vi "Parameter selection.vi"(2 "Selected Channel":i32(listbox), 5 "Hc0 2":i32(listbox), 7 "默认":bool=TRUE, 10 "全部结构组":T1[](array[typedef]), 11 "逻辑通道组":i32[](array[numeric])) -> (0 "subarray":string[](array[string]), 1 "改变？":bool, 3 "通道组":i32[](array[numeric]), 4 "Array 2":string[](array[string]))   [LabVIEW 2025]
uses:
  data structure.ctl
panel:
  out "Array 6":string[](array[string])
  out "Array":string[](array[string])
  out "subarray 4":string[](array[string])
  out "subarray 3":string[](array[string])
  out "deleted portion":string[](array[string])
  out "subarray 2":string[](array[string])
  out "Array 5":string[][](array[string])
  out "array w/ subset deleted":string[][](array[string])
  out "Array 4":string[](array[string])
  out "Array 3":string[](array[string])
  out "Item Names 2":string[][](array[string])
  in  "数据列表 2":enum32{"40TR", "Chiller"}(tab)
  in  "Hc1 2":i32(listbox)
  in  "数据列表":enum32{"40TR", "Chiller"}(tab)
  in  "Hc0":i32(listbox)
  in  "Hc1":i32(listbox)
  out "Item Names":string[][](array[string])
  in  "取消按钮":bool
  in  "确定按钮":bool
  in  "向下按钮":bool
  in  "向上按钮":bool
  in  "删除按钮":bool
  in  "添加按钮":bool
  in  "All Channel":i32(listbox)
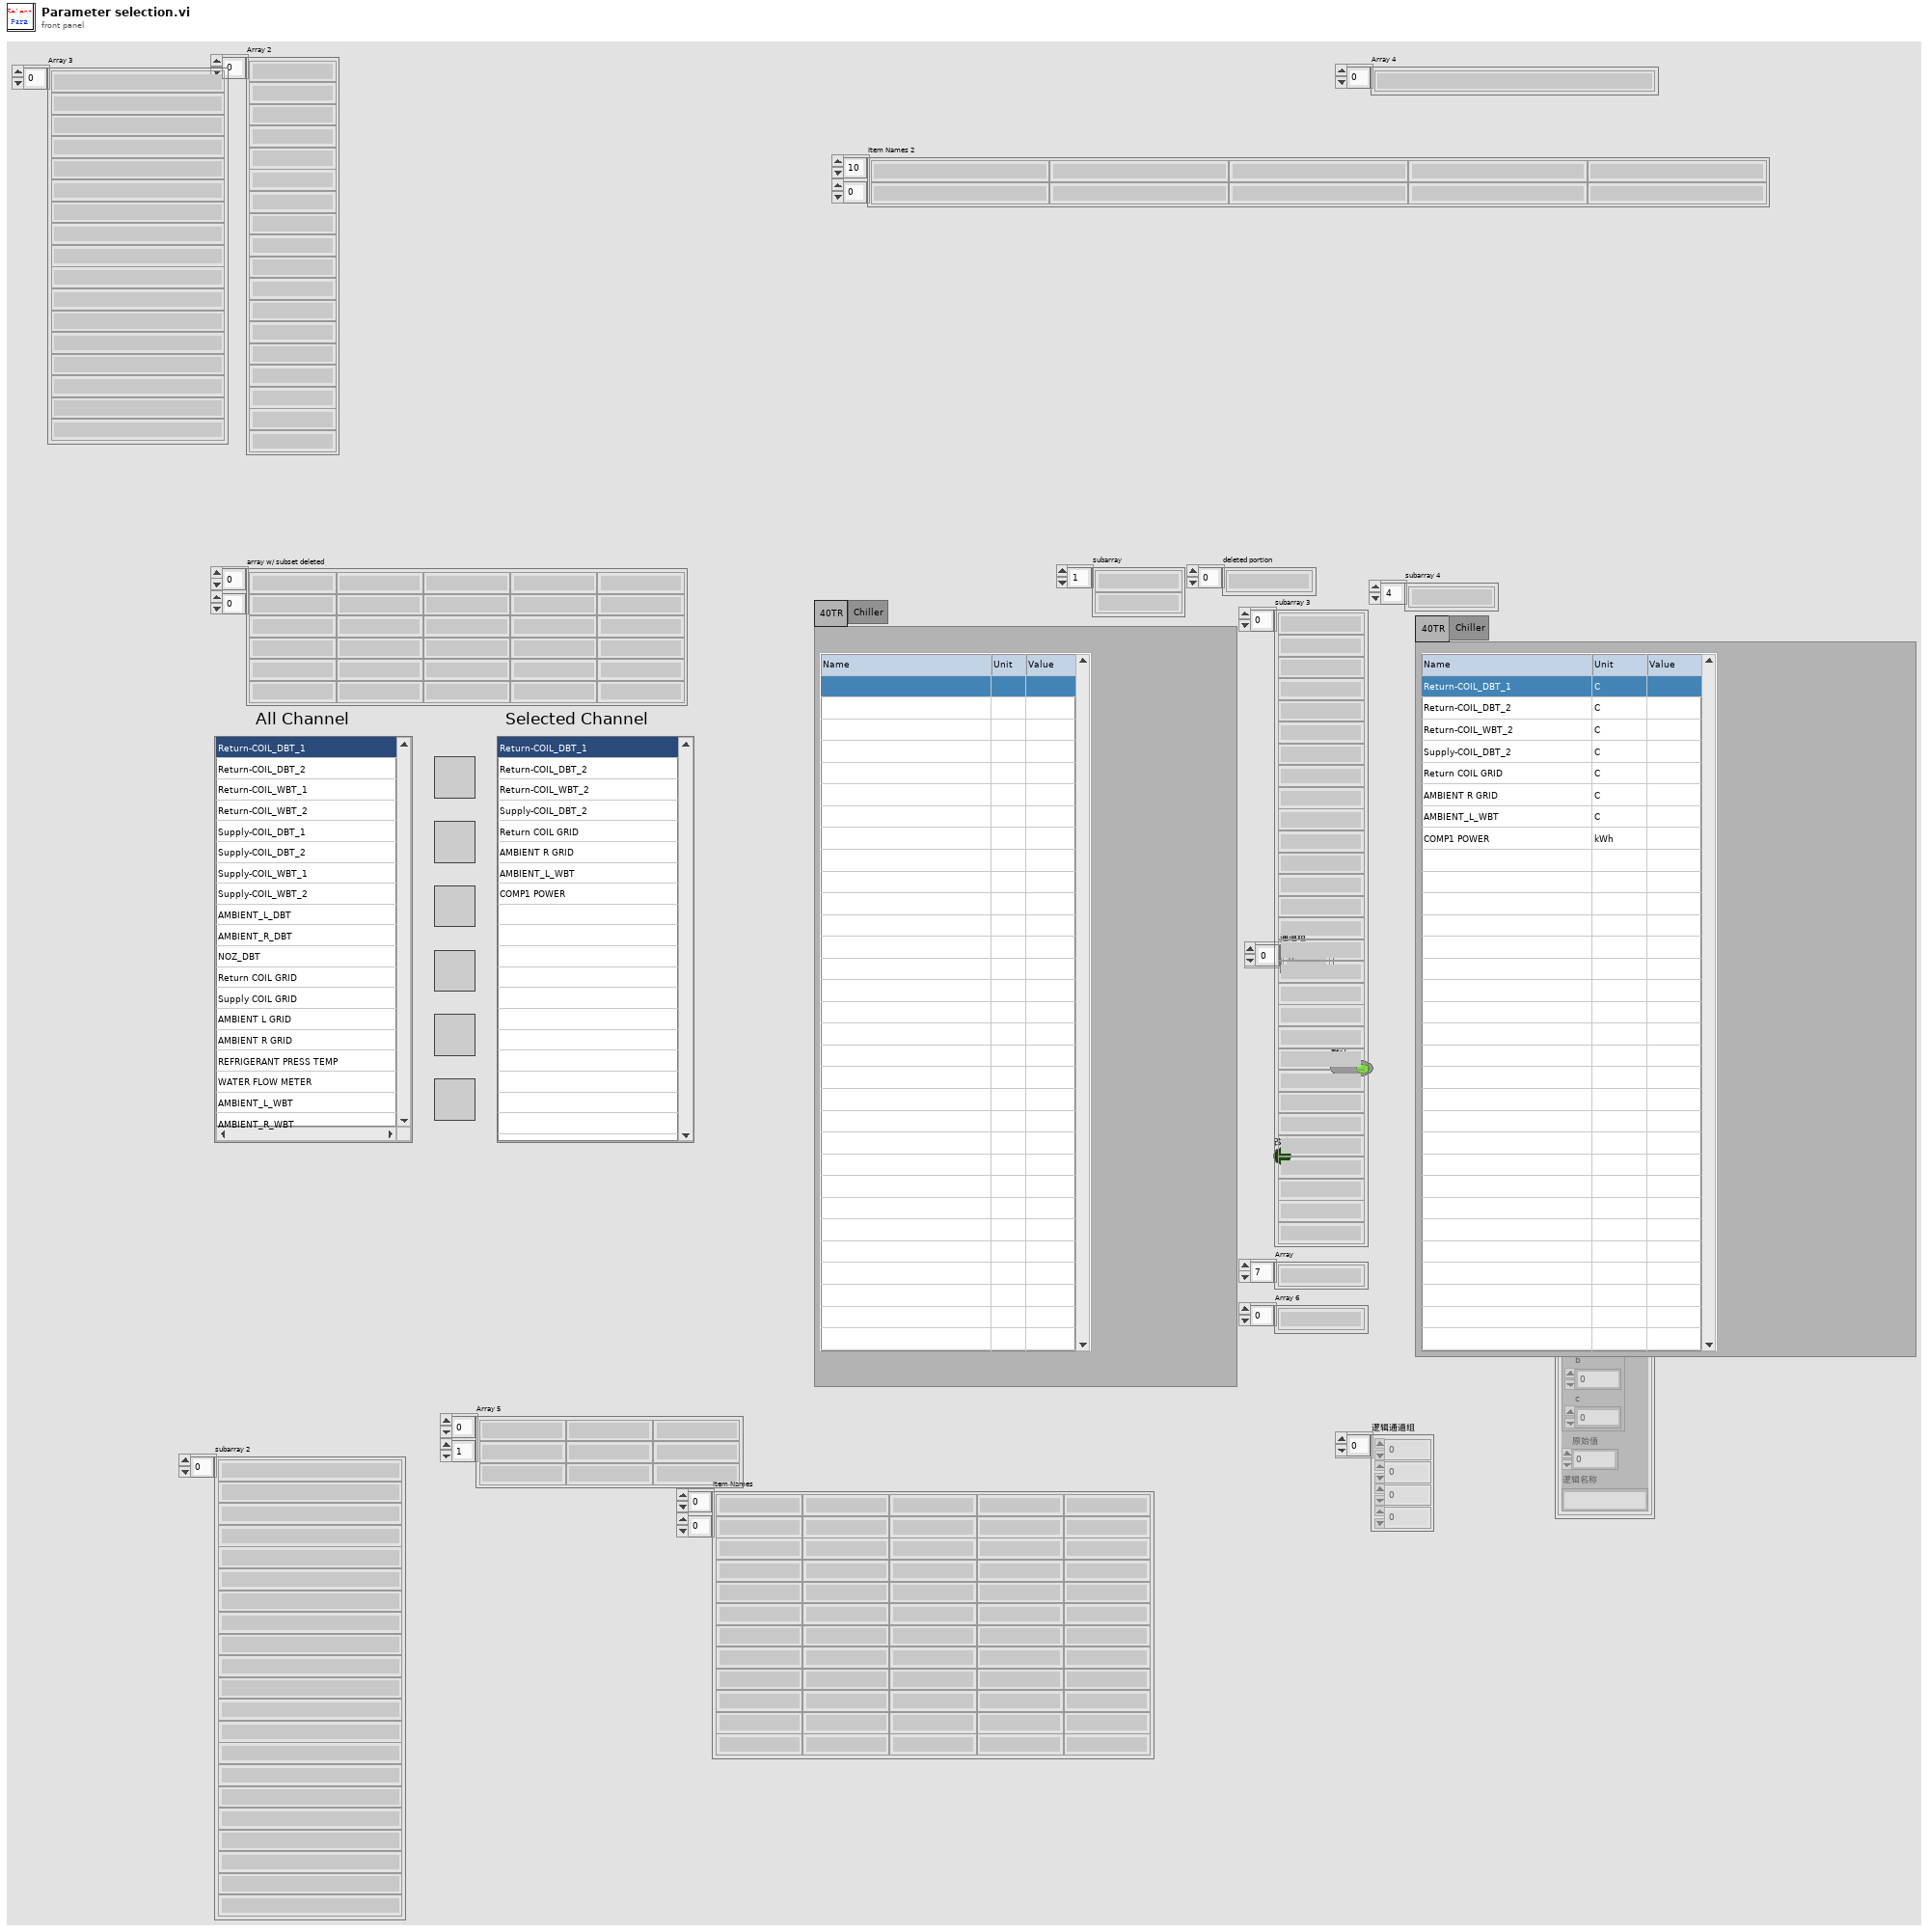
[diagram p1: front panel]
types:
  T1 = typedef "data structure.ctl" = cluster{"展示名称":string, "单位":string, "值":string, "物理通道":i32, "逻辑通道":i32, "小数点":i16, "数值":dbl, "修正因子":cluster{"a":dbl, "b":dbl, "c":dbl}, "原始值":sgl, "逻辑名称":string}
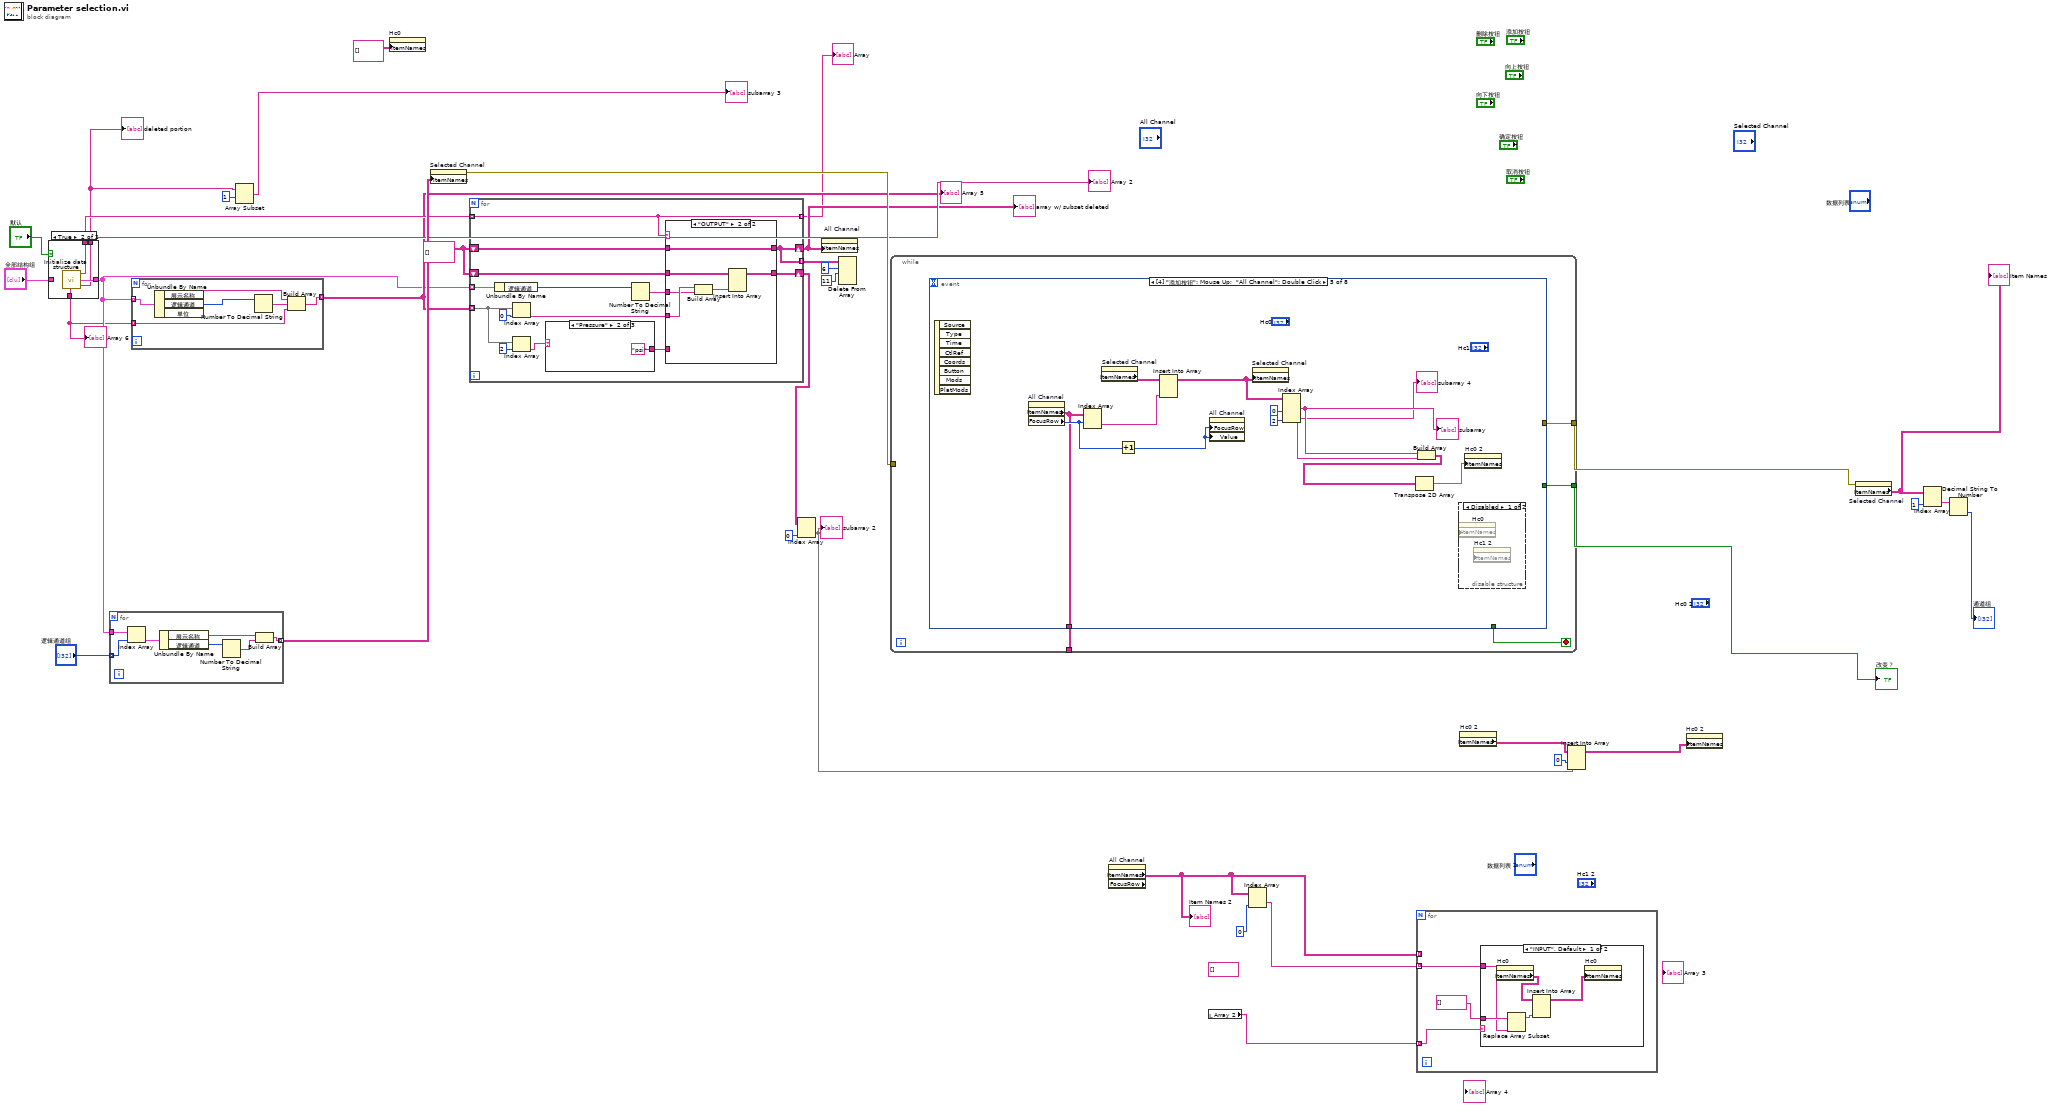
[diagram p0: block diagram]
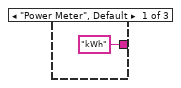
[diagram p2: hidden frame]
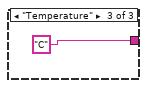
[diagram p3: hidden frame]
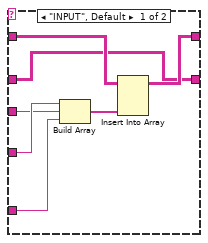
[diagram p4: hidden frame]
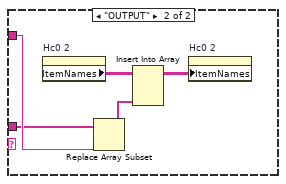
[diagram p5: hidden frame]
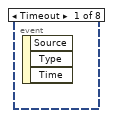
[diagram p6: hidden frame]
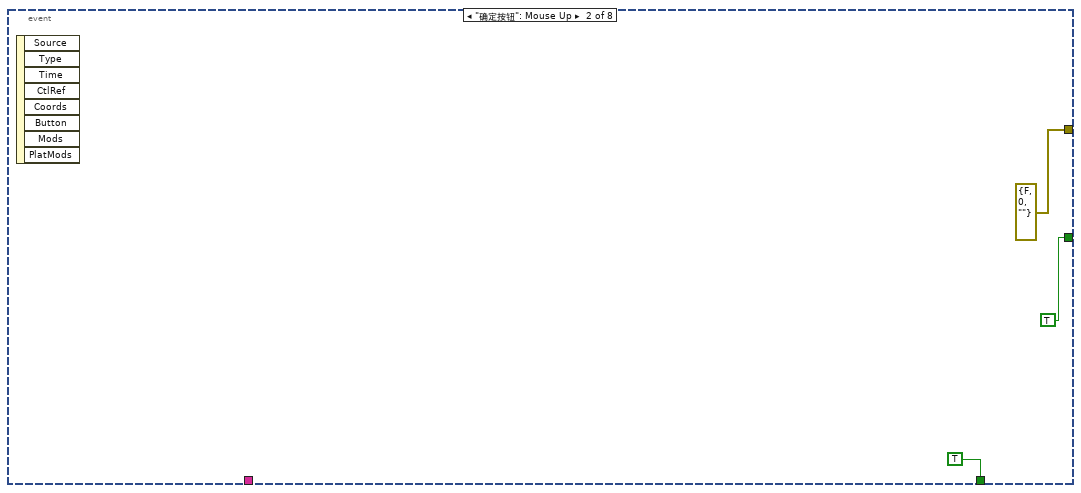
[diagram p7: hidden frame]
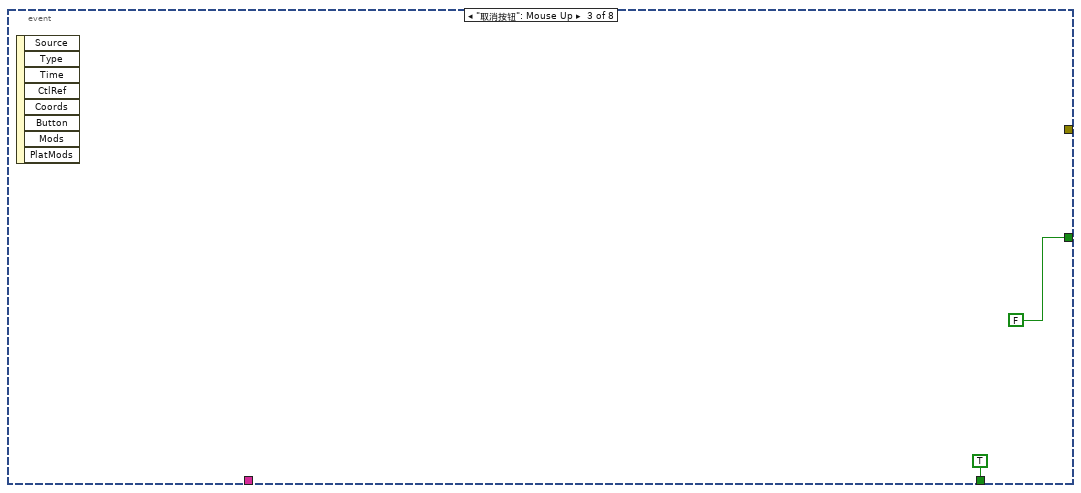
[diagram p8: hidden frame]
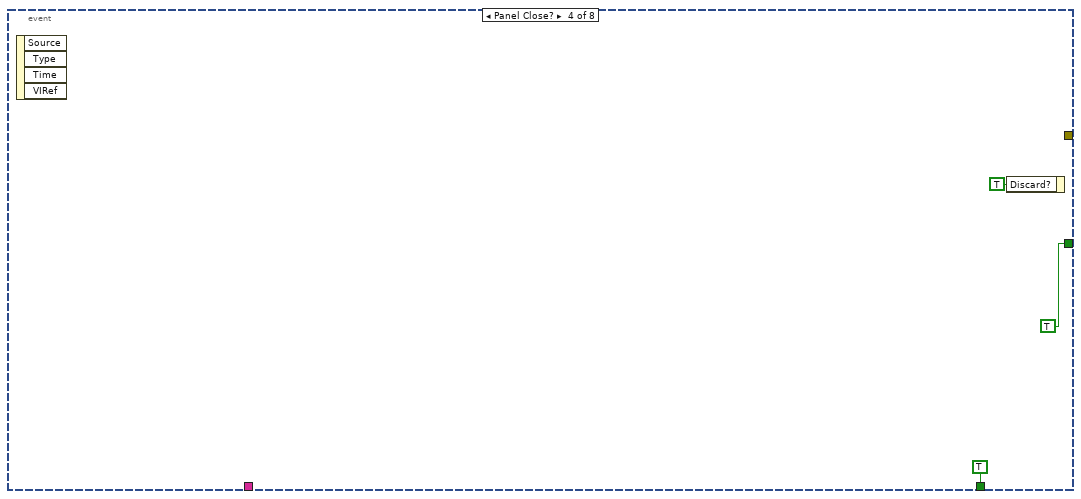
[diagram p9: hidden frame]
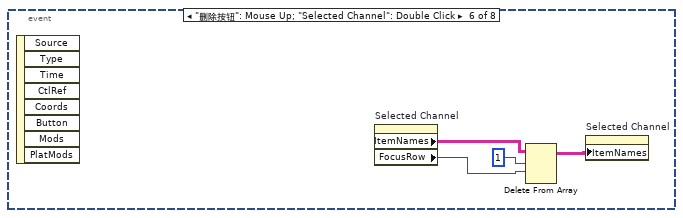
[diagram p11: hidden frame]
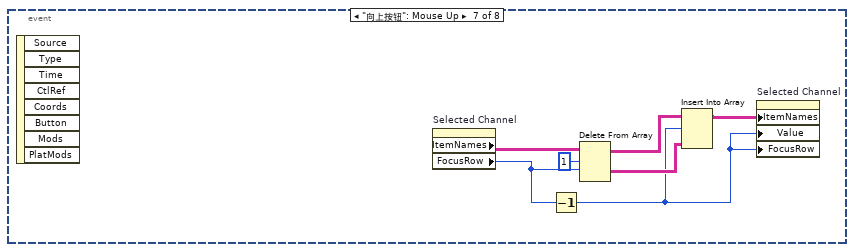
[diagram p12: hidden frame]
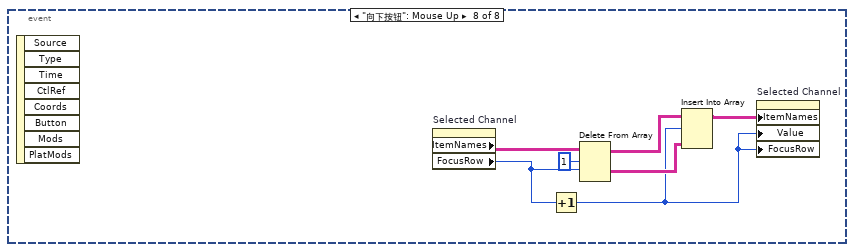
[diagram p13: hidden frame]
diagram:
  w13 = string[][] []
  (unwired) string[] []
  n1 = case shown="True" "默认" {
    tunnel: "全部结构组" -> [w36 _]
    tunnel: [w36 w40] -> w15
    tunnel: [_ w39] -> w19
    tunnel: [_ w38] -> w6
    tunnel: [_ w37] -> w2
    frame False {
    }
    frame True {
      n2 = call "Initialize data structure.vi"() -> ("Array 2"=w37:string[], "Array"=w39:string[], "数据结构组"=w40:T1[], "deleted portion"=w38:string[])  [unwired: 5 in]
    }
  }
  "Array 2" <- w19
  "deleted portion" <- w6
  "Array 6" <- w2
  n3 = for {
    tunnel: w15 -> [w47]
    tunnel: "逻辑通道组" -> [w46] mode=indexing
    tunnel: [w41] -> w25 mode=indexing
    n4 = Index Array(array=w47, index=w46) -> (element=w45:T1)
    n5 = Unbundle By Name(w45) -> ("展示名称"=w43:string, "逻辑通道"=w42:i32)
    n6 = Number To Decimal String(number=w42) -> (decimal integer string=w44:string)  [unwired: 1 in]
    n7 = Build Array(w43, w44) -> (w41:string[])
  }
  n8 = for {
    tunnel: w15 -> [w53] mode=indexing
    tunnel: [w49] -> w16 mode=indexing
    tunnel: w2 -> [w48] mode=indexing
    n9 = Unbundle By Name(w53) -> ("展示名称"=w50:string, "逻辑通道"=w52:i32)  [unwired: 1 out]
    n10 = Number To Decimal String(number=w52) -> (decimal integer string=w51:string)  [unwired: 1 in]
    n11 = Build Array(w50, w51, w48) -> (w49:string[])
  }
  "Array 5" <- w16
  n12 = Array Subset(array=w6, index=1) -> (→"subarray 3":string[])  [unwired: 1 in]
  n13 = property on="Hc0" class="MCListbox (strict)"("ItemNames"=string[][] [] ("Item Names")) -> ()  [unwired: 2 in, 2 out]
  n14 = property on="Selected Channel" class="MCListbox (strict)"("ItemNames"=w25) -> (error out=w26:errorcluster)  [unwired: 2 in, 1 out]
  n15 = for {
    tunnel: [w67] -> w3 mode=indexing
    tunnel: w19 -> [w67] mode=indexing
    tunnel: w16 -> [w57] mode=indexing
    shift-right: [w64] -> w14
    shift-left: w13 -> [w66]
    tunnel: [w64] -> w17 mode=indexing
    tunnel: w15 -> [w62] mode=indexing
    shift-right: [w58] -> w11
    shift-left: w13 -> [w59]
    n16 = Unbundle By Name(w62) -> ("逻辑通道"=w61:i32)
    n17 = Index Array(array=w57, index=0) -> (element=w65:string)
    n18 = Index Array(array=w57, index=2) -> (element=w55:string)
    n19 = case shown="\"Pressure\"" w55 {
      tunnel: ["kWh" ("单位") "psi" ("单位") "C" ("单位")] -> w54
      frame "Power Meter", Default {
      }
      frame "Pressure" {
      }
      frame "Temperature" {
      }
    }
    n20 = Number To Decimal String(number=w61) -> (decimal integer string=w60:string)  [unwired: 1 in]
    n21 = case shown="\"OUTPUT\"" w67 {
      tunnel: w66 -> [w77 w83]
      tunnel: w65 -> [w75 w82]
      tunnel: [w76 w83] -> w64
      tunnel: w60 -> [w74 w81]
      tunnel: w59 -> [w72 w79]
      tunnel: [w72 w78] -> w58
      tunnel: w54 -> [w71 _]
      frame "INPUT", Default {
        n22 = Build Array(w75, w74, w71) -> (w73:string[])
        n23 = Insert Into Array(array=w77, new element=w73) -> (w76:string[][])  [unwired: 2 in]
      }
      frame "OUTPUT" {
        n24 = Build Array(w82, w81) -> (w80:string[])
        n25 = Insert Into Array(array=w79, new element=w80) -> (w78:string[][])  [unwired: 2 in]
      }
    }
  }
  "array w/ subset deleted" <- w14
  "Array" <- w3
  n26 = Index Array(array=w11, index (col)=0 ("disabled index (col)")) -> (element=w9:string[])  [unwired: 1 in]
  "subarray 2" <- w9
  n27 = property on="All Channel" class="MCListbox (strict)"("ItemNames"=w14) -> ()  [unwired: 2 in, 2 out]
  n28 = Delete From Array(array=w17, length=6, index (dim 0)=11 ("index (row)")) -> ()  [unwired: 2 in, 2 out]
  n29 = while {
    tunnel: [w86] -> w32
    tunnel: [w85] -> w31
    tunnel: w26 -> [_]
    tunnel: [w84] -> _
    stop <- w87 stop-if-true
    n30 = event shown="[4] \"添加按钮\": Mouse Up;  \"All Channel\": Double Click" {
      selector: _ -> [_ _ _ _ _ _ _ _]
      dyn-events: _ -> [_ _ _ _ _ _ _ _]
      timeout: _ -> [_ _ _ _ _ _ _ _]
      tunnel: [_ TRUE TRUE TRUE _ _ _ _] -> w87
      tunnel: [_ TRUE FALSE TRUE _ _ _ _] -> w86
      tunnel: [_ errorcluster {"status"=FALSE, "code"=0, "source"=""} ("错误常量") _ _ _ _ _ _] -> w85
      tunnel: [_ _ _ _ w103 _ _ _] -> w84
      event Timeout {
        n31 = event-data() -> ()  [unwired: 1 in, 3 out]
      }
      event "确定按钮": Mouse Up {
        n32 = event-data() -> ()  [unwired: 1 in, 8 out]
      }
      event "取消按钮": Mouse Up {
        n33 = event-data() -> ()  [unwired: 1 in, 8 out]
      }
      event Panel Close? {
        n34 = event-data() -> ()  [unwired: 1 in, 4 out]
        n35 = event-data("Discard?"=TRUE ("放弃？")) -> ()  [unwired: 1 in, 1 out]
      }
      event "添加按钮": Mouse Up; "All Channel": Double Click {
        n36 = event-data() -> ()  [unwired: 1 in, 8 out]
        n37 = property on="All Channel" class="MCListbox (strict)"() -> ("ItemNames"=w103:string[][], "FocusRow"=w105:i32)  [unwired: 2 in, 2 out]
        n38 = Index Array(array=w103, index (row)=w105) -> (element=w106:string[])  [unwired: 1 in]
        n39 = property on="Selected Channel" class="MCListbox (strict)"() -> ("ItemNames"=w107:string[][])  [unwired: 2 in, 2 out]
        n40 = Increment(x=w105) -> (x+1=w104:i32)
        n41 = Insert Into Array(array=w107, new element=w106) -> (w102:string[][])  [unwired: 2 in]
        n42 = property on="All Channel" class="MCListbox (strict)"("FocusRow"=w104, "Value"=w104) -> ()  [unwired: 2 in, 2 out]
        n43 = property on="Selected Channel" class="MCListbox (strict)"("ItemNames"=w102) -> ()  [unwired: 2 in, 2 out]
        n44 = Index Array(array=w102, index (col) #1=0 ("disabled index (col)"), index (col) #2=2 ("index (col)")) -> (element #1=w99:string[], element #2=w98:string[])  [unwired: 2 in]
        "subarray" <- w99
        "subarray 4" <- w98
        n45 = Build Array(w99, w98) -> (w97:string[][])
        n46 = Transpose 2D Array(2D array=w97) -> (transposed array=w96:string[][])
        n47 = disable-structure shown="Disabled" {
          frame Disabled {
            n48 = property on="Hc0" class="MCListbox (strict)" props=["ItemNames"]() -> ()  [unwired: 3 in, 2 out]
            n49 = property on="Hc1 2" class="MCListbox (strict)" props=["ItemNames"]() -> ()  [unwired: 3 in, 2 out]
          }
          frame Enabled {
          }
        }
        n50 = property on="Hc0 2" class="MCListbox (strict)"("ItemNames"=w96) -> ()  [unwired: 2 in, 2 out]
      }
      event "删除按钮": Mouse Up; "Selected Channel": Double Click {
        n51 = event-data() -> ()  [unwired: 1 in, 8 out]
        n52 = property on="Selected Channel" class="MCListbox (strict)"() -> ("ItemNames"=w111:string[][], "FocusRow"=w109:i32)  [unwired: 2 in, 2 out]
        n53 = Delete From Array(array=w111, length=1 ("长度"), index (row)=w109) -> (array with subset deleted=w108:string[][])  [unwired: 1 in, 1 out]
        n54 = property on="Selected Channel" class="MCListbox (strict)"("ItemNames"=w108) -> ()  [unwired: 2 in, 2 out]
      }
      event "向上按钮": Mouse Up {
        n55 = event-data() -> ()  [unwired: 1 in, 8 out]
        n56 = property on="Selected Channel" class="MCListbox (strict)"() -> ("ItemNames"=w118:string[][], "FocusRow"=w116:i32)  [unwired: 2 in, 2 out]
        n57 = Decrement(x=w116) -> (x-1=w112:i32)
        n58 = Delete From Array(array=w118, length=1 ("长度"), index (row)=w116) -> (deleted portion=w114:string[][], array with subset deleted=w115:string[][])  [unwired: 1 in]
        n59 = Insert Into Array(array=w115, index (row)=w112, new element=w114) -> (w113:string[][])  [unwired: 1 in]
        n60 = property on="Selected Channel" class="MCListbox (strict)"("ItemNames"=w113, "Value"=w112, "FocusRow"=w112) -> ()  [unwired: 2 in, 2 out]
      }
      event "向下按钮": Mouse Up {
        n61 = event-data() -> ()  [unwired: 1 in, 8 out]
        n62 = property on="Selected Channel" class="MCListbox (strict)"() -> ("ItemNames"=w125:string[][], "FocusRow"=w123:i32)  [unwired: 2 in, 2 out]
        n63 = Increment(x=w123) -> (x+1=w119:i32)
        n64 = Delete From Array(array=w125, length=1 ("长度"), index (row)=w123) -> (deleted portion=w121:string[][], array with subset deleted=w122:string[][])  [unwired: 1 in]
        n65 = Insert Into Array(array=w122, index (row)=w119, new element=w121) -> (w120:string[][])  [unwired: 1 in]
        n66 = property on="Selected Channel" class="MCListbox (strict)"("ItemNames"=w120, "Value"=w119, "FocusRow"=w119) -> ()  [unwired: 2 in, 2 out]
      }
    }
  }
  "改变？" <- w32
  n67 = property on="All Channel" class="MCListbox (strict)" props=["ItemNames", "FocusRow"]() -> ("ItemNames"=w23:string[][])  [unwired: 2 in, 3 out]
  "Item Names 2" <- w23
  n68 = local read "Array 2"() -> (w24:string[])
  n69 = Index Array(array=w23, index (col)=0 ("disabled index (col)")) -> (element=w21:string[])  [unwired: 1 in]
  n70 = for {
    tunnel: w23 -> [_] mode=indexing
    tunnel: w24 -> [w128] mode=indexing
    tunnel: w21 -> [w127] mode=indexing
    n71 = case shown="\"INPUT\", Default" w128 {
      tunnel: w127 -> [w132 w135]
      tunnel: string[] [] ("new element/subarray") -> [w133 w134]
      frame "INPUT", Default {
        n72 = property on="Hc0" class="MCListbox (strict)"() -> ("ItemNames"=w130:string[][])  [unwired: 2 in, 2 out]
        n73 = Replace Array Subset(array=w133, new element=w132) -> (w131:string[])  [unwired: 1 in]
        n74 = Insert Into Array(array=w130, new element=w131) -> (w129:string[][])  [unwired: 2 in]
        n75 = property on="Hc0" class="MCListbox (strict)"("ItemNames"=w129) -> ()  [unwired: 2 in, 2 out]
      }
      frame "OUTPUT" {
        n76 = property on="Hc0 2" class="MCListbox (strict)"() -> ("ItemNames"=w138:string[][])  [unwired: 2 in, 2 out]
        n77 = Replace Array Subset(array=w134, new element=w135) -> (w136:string[])  [unwired: 1 in]
        n78 = Insert Into Array(array=w138, new element=w136) -> (w137:string[][])  [unwired: 2 in]
        n79 = property on="Hc0 2" class="MCListbox (strict)"("ItemNames"=w137) -> ()  [unwired: 2 in, 2 out]
      }
    }
  }
  n80 = property on="Hc0 2" class="MCListbox (strict)"() -> ("ItemNames"=w10:string[][])  [unwired: 2 in, 2 out]
  n81 = Insert Into Array(array=w10, index (col)=0 ("disabled index (col)"), new element=w9) -> (w8:string[][])  [unwired: 1 in]
  n82 = property on="Hc0 2" class="MCListbox (strict)"("ItemNames"=w8) -> ()  [unwired: 2 in, 2 out]
  n83 = property on="Selected Channel" class="MCListbox (strict)"(error in=w31) -> ("ItemNames"=w30:string[][])  [unwired: 1 in, 2 out]
  "Item Names" <- w30
  n84 = Index Array(array=w30, index (col)=1 ("禁用的索引 (列)")) -> (element=w28:string[])  [unwired: 1 in]
  n85 = Decimal String To Number(string=w28) -> (number=→"通道组":i32[])  [unwired: 2 in, 1 out]
